vi "Test Encode Decode.vi"() -> ()   [LabVIEW 2021]
uses:
  typedef/Relay ID.ctl
  USB Relay Control.lvlib
panel:
  out "pass":bool
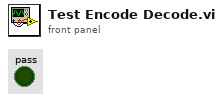
[diagram p1: front panel]
types:
  T1 = typedef "USB Relay Control.lvlib/Relay ID.ctl" = cluster{"Vendor ID":u8, "Product ID":u8, "Serial Number":u32, "Submodule ID":u8}
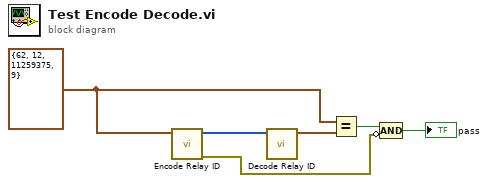
[diagram p0: block diagram]
diagram:
  w4 = T1 {"Vendor ID"=62, "Product ID"=12, "Serial Number"=11259375, "Submodule ID"=9} ("Relay ID")
  n1 = call "Encode Relay ID.vi"("Relay ID"=w4) -> ("error out"=w1:errorcluster, "Encoded ID"=w6:u8[])  [unwired: 9 in]
  n2 = call "Decode Relay ID.vi"("Encoded ID"=w6) -> ("Relay ID"=w5:T1)  [unwired: 10 in]
  n3 = Equal?(x=w4, y=w5) -> (x = y?=w3:bool)
  n4 = Compound Arithmetic op=AND(w3, invert w1) -> (→"pass":bool)
